vi "mS Wait Until.vi"(9 "mS Delta":u16, 11 "mS Start Time":u32) -> (1 "Done":bool, 3 "mS End Time":u32)   [LabVIEW 2013]
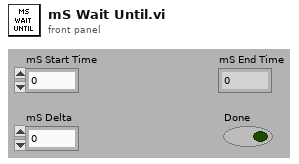
[diagram p1: front panel]
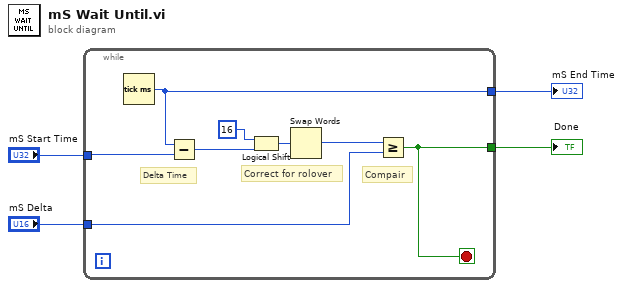
[diagram p0: block diagram]
diagram:
  n1 = while {
    tunnel: [w11] -> w2
    tunnel: "mS Delta" -> [w12]
    tunnel: "mS Start Time" -> [w10]
    tunnel: [w9] -> w4
    stop <- w11 stop-if-true
    # "Compair"
    # "Delta Time"
    # "Correct for rolover"
    n2 = Tick Count (ms)() -> (millisecond timer value=w9:u32)
    n3 = Subtract(x=w9, y=w10) -> (x-y=w6:u32)
    n4 = Logical Shift(y=i8 16, x=w6) -> (x << y=w7:u32)
    n5 = Swap Words(1:w7) -> (0:w5:u32)
    n6 = Greater Or Equal?(x=w5, y=w12) -> (x >= y?=w11:bool)
  }
  "mS End Time" <- w4
  "Done" <- w2
